vi "Read Light Spectrum.vi"(8 "error in (no error)":errorcluster, 11 "Light Spectrum in":refnum<class "I2C Light Spectrum Sensor.lvclass">) -> (0 "error out":errorcluster, 2 "Light Spectrum":dbl[](array[numeric]), 3 "Light Spectrum out":refnum<class "I2C Light Spectrum Sensor.lvclass">)   [LabVIEW 2020, in "CTI-Peripheral.lvlib" / "I2C Light Spectrum Sensor.lvclass"]
uses:
  I2C Light Spectrum Sensor.lvclass
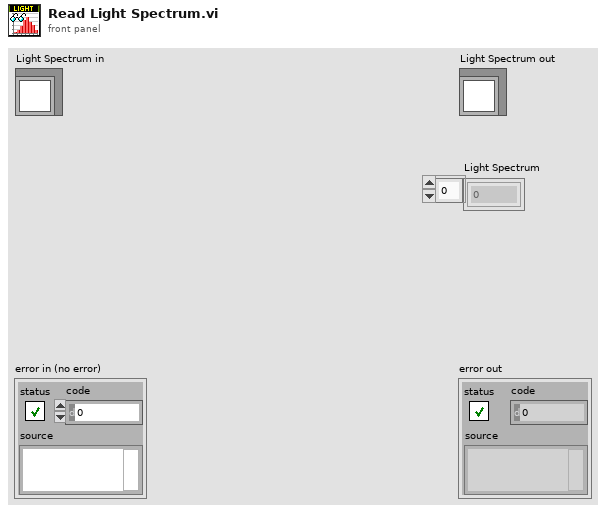
[diagram p1: front panel]
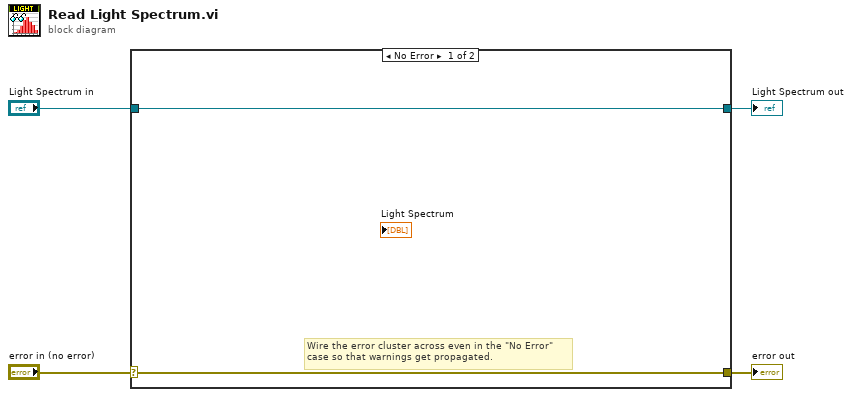
[diagram p0: block diagram]
diagram:
  n1 = case shown="No Error" "error in (no error)" {
    selector: "error in (no error)" -> [w5 w8]
    tunnel: [w5 w8] -> w3
    tunnel: [w6 w7] -> w1
    tunnel: "Light Spectrum in" -> [w6 w7]
    frame No Error {
      # "Wire the error cluster across even in the \"No Error\"\ncase so that warnings get propagated."
    }
    frame Error {
    }
  }
  "error out" <- w3
  "Light Spectrum out" <- w1
